vi "VIH - CHM Project - Get HTML Paths and Default Topic.vi"(9 "HHP_Generation":T3={"HHP_Template"=enum."default", "HHP_Template_CustomPath"=path "", "HHP_Target"=enum."default", "HHP_Target_CustomPath"=path "", "HHP_CreateTOC"=TRUE, "HHP_CreateIDX"=TRUE, "HHP_DefaultTopic"=enum."auto", "HHP_DefaultTopic_CustomPath"=path "", "CHM_Filename"=path "", "HHP_AutoBuild"=FALSE, "CHM_AutoBuild"=FALSE}, 11 "Project Files":T2) -> (1 "Default Topic file":path, 3 "HTML Files":path[](array[path]))   [LabVIEW 2014]
doc: "::: VI Helpeks :::\nCopyright (c) 2000-2026 Konstantin Shifershteyn. All rights reserved."
uses:
  VIH - CHM Project - HHP Generation Params Cluster.ctl
  _VIH HelpGen - Palette.llb/VIH HelpGen Typedef - Palette - Item Type Enum.ctl
panel:
  # "VI Helpeks\nCopyright (c) 2012-2026 Konstantin Shifershteyn"
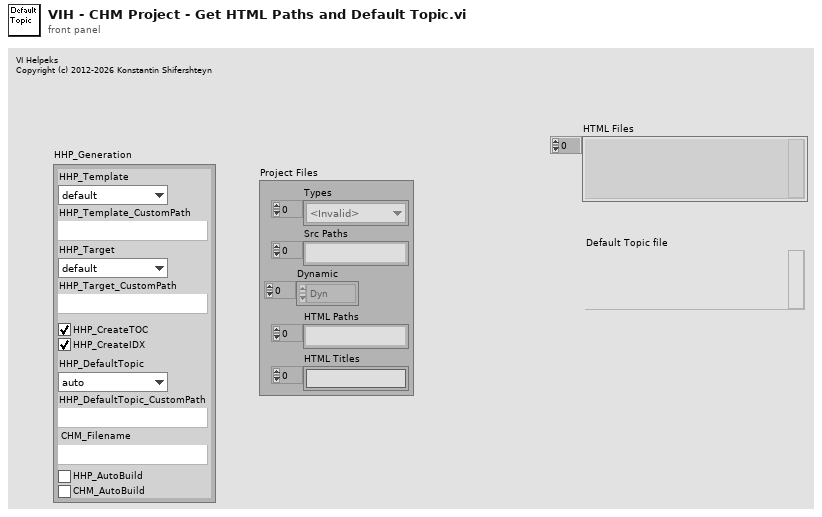
[diagram p1: front panel]
types:
  T1 = typedef "VIH HelpGen Typedef - Palette - Item Type Enum.ctl" = enum32{"<Invalid>", "<unknown>", "VI", "Menu", "LV Func", "Express VI", "Poly VI", "CTL", "HTML"}
  T2 = cluster{"Types":T1[], "Src Paths":path[], "Dynamic":enum16{"Dyn", "Stat", "Both"}[], "HTML Paths":path[], "HTML Titles":string[]}
  T3 = typedef "VIH - CHM Project - HHP Generation Params Cluster.ctl" = cluster{"HHP_Template":enum16{"default", "custom"}, "HHP_Template_CustomPath":path, "HHP_Target":enum16{"default", "custom"}, "HHP_Target_CustomPath":path, "HHP_CreateTOC":bool, "HHP_CreateIDX":bool, "HHP_DefaultTopic":enum16{"auto", "custom"}, "HHP_DefaultTopic_CustomPath":path, "CHM_Filename":path, "HHP_AutoBuild":bool, "CHM_AutoBuild":bool}
  T4 = cluster{"Item/File Type":T1, enum16{"Dyn", "Stat", "Both"}}[]
  T5 = cluster{"Item/File Type":T1, enum16{"Dyn", "Stat", "Both"}}
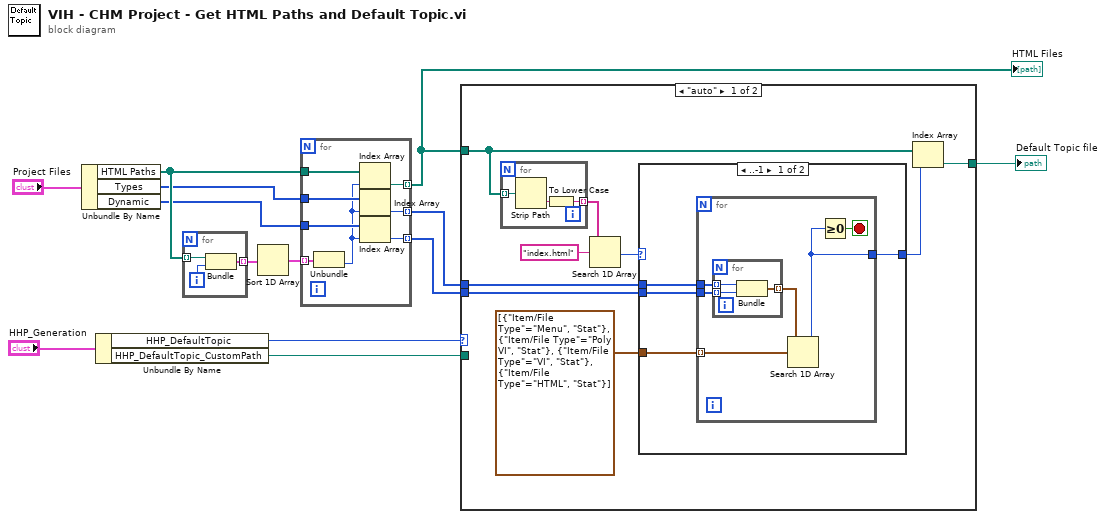
[diagram p0: block diagram]
diagram:
  n1 = Unbundle By Name("Project Files") -> ("HTML Paths"=w7:path[], "Types"=w6:T1[], "Dynamic"=w5:enum16{"Dyn", "Stat", "Both"}[])
  n2 = Unbundle By Name("HHP_Generation") -> ("HHP_DefaultTopic"=w12:enum16{"auto", "custom"}, "HHP_DefaultTopic_CustomPath"=w13:path)
  n3 = for {
    tunnel: w7 -> [w16] mode=indexing
    tunnel: [w14] -> w8 mode=indexing
    i -> [w15]
    n4 = Bundle(w16, w15) -> (w14:cluster{path, i32})  [unwired: 1 in]
  }
  n5 = Sort 1D Array(array=w8) -> (sorted array=w4:cluster{path, i32}[])
  n6 = for {
    tunnel: w7 -> [w24]
    tunnel: w6 -> [w23]
    tunnel: w5 -> [w22]
    tunnel: w4 -> [w21] mode=indexing
    tunnel: [w19] -> w3 mode=indexing
    tunnel: [w18] -> w2 mode=indexing
    tunnel: [w17] -> w1 mode=indexing
    n7 = Unbundle(w21) -> (w20:i32)  [unwired: 1 out]
    n8 = Index Array(array=w24, index=w20) -> (element=w19:path)
    n9 = Index Array(array=w23, index=w20) -> (element=w18:T1)
    n10 = Index Array(array=w22, index=w20) -> (element=w17:enum16{"Dyn", "Stat", "Both"})
  }
  "HTML Files" <- w3
  n11 = case shown="\"auto\"" w12 {
    tunnel: w2 -> [w33 _]
    tunnel: w1 -> [w32 _]
    tunnel: w3 -> [w29 _]
    tunnel: [w28 w51] -> w9
    tunnel: w13 -> [_ w51]
    frame "auto" {
      n12 = for {
        tunnel: w29 -> [w50] mode=indexing
        tunnel: [w48] -> w31 mode=indexing
        n13 = Strip Path(path=w50) -> (name=w49:string)  [unwired: 1 out]
        n14 = To Lower Case(string=w49) -> (all lower case string=w48:string)
      }
      n15 = Search 1D Array(1D array=w31, element="index.html") -> (index of element=w26:i32)  [unwired: 1 in]
      n16 = case shown="..-1" w26 {
        selector: w26 -> [_ w47]
        tunnel: w33 -> [w37 _]
        tunnel: w32 -> [w36 _]
        tunnel: [w35 w47] -> w27
        tunnel: T4 [{"Item/File Type"=enum."Menu", enum."Stat"}, {"Item/File Type"=enum."Poly VI", enum."Stat"}, {"Item/File Type"=enum."VI", enum."Stat"}, {"Item/File Type"=enum."HTML", enum."Stat"}] -> [w34 _]
        frame ..-1 {
          n17 = for {
            tunnel: w37 -> [w43]
            tunnel: w36 -> [w42]
            tunnel: [w40] -> w35
            tunnel: w34 -> [w38] mode=indexing
            stop <- w39 stop-if-true
            n18 = for {
              tunnel: w43 -> [w46] mode=indexing
              tunnel: w42 -> [w45] mode=indexing
              tunnel: [w44] -> w41 mode=indexing
              n19 = Bundle("Item/File Type"=w46, w45) -> (w44:T5)  [unwired: 1 in]
            }
            n20 = Search 1D Array(1D array=w41, element=w38) -> (index of element=w40:i32)  [unwired: 1 in]
            n21 = Greater Or Equal To 0?(x=w40) -> (x >= 0?=w39:bool)
          }
        }
        frame 0.. {
        }
      }
      n22 = Index Array(array=w29, index=w27) -> (element=w28:path)
    }
    frame "custom" {
    }
  }
  "Default Topic file" <- w9
